vi "ControllerUI_New - 副本.vi"() -> ()   [LabVIEW 2026]
uses:
  <vilib>/Utility/error.llb/Trim Whitespace One-Sided.vi
panel:
  in  "Tab Control":T1(tab)
  out "background 2":picture
  in  "5-Day Rainstorm-to-Flood":bool
  out "script Status":string
  in  "voltage 1":dbl
  in  "DESD4 SOC":dbl(slide) step=1.0 scale=0.0..100.0 scale format="%#.6g"
  in  "DESD3 SOC":dbl(slide) step=1.0 scale=0.0..100.0 scale format="%#.6g"
  in  "DESD2 SOC":dbl(slide) step=1.0 scale=0.0..100.0 scale format="%#.6g"
  in  "wind speed":dbl(knob) caption="Wind Speed (m/s)" min=0.0 max=30.0 step=0.5 scale=0.0..255.0
  in  "stop":bool
  in  "Send UDP Command":bool caption="IO Building Send"
  out "Device Badge":string
  out "Selected Summary":string
  out "Device Description":string
  out "Device Name":string
  in  "DESD1 SOC":dbl(slide) step=1.0 scale=0.0..100.0 scale format="%#.6g"
  in  "BTN_DESD_4":bool
  in  "BTN_PV_1":bool
  in  "BTN_DESD_2":bool
  in  "BTN_Gen_1":bool
  in  "BTN_DESD_1":bool
  in  "BTN_Gen_2":bool
  in  "BTN_DESD_3":bool
  in  "BTN_PV_2":bool
  in  "BTN_Load_2":bool
  in  "BTN_Load_4":bool
  in  "BTN_Grid_1":bool
  in  "BTN_Load_3":bool
  in  "BTN_Wind_Turbine":bool
  out "background":picture
  in  "IO 1":bool
  in  "IO 2":bool
  in  "IO 3":bool
  in  "IO 4":bool
  in  "IO 6":bool
  in  "IO 7":bool
  in  "IO 8":bool
  in  "IO 5":bool
  in  "IO 9":bool
  in  "IO 10":bool
  in  "IO 11":bool
  in  "IO 12":bool
  in  "IO 13":bool
  in  "IO 14":bool
  in  "IO 15":bool
  in  "IO 16":bool
  in  "voltage 2":dbl
  in  "voltage 3":dbl
  in  "voltage 4":dbl
  # "LabVIEW-Based Physical Sandbox Intelligent Control System"
  # "LabVIEW-Based Physical Sandbox Intelligent Control System"
  # "Node Information"
  # "Control Panel"
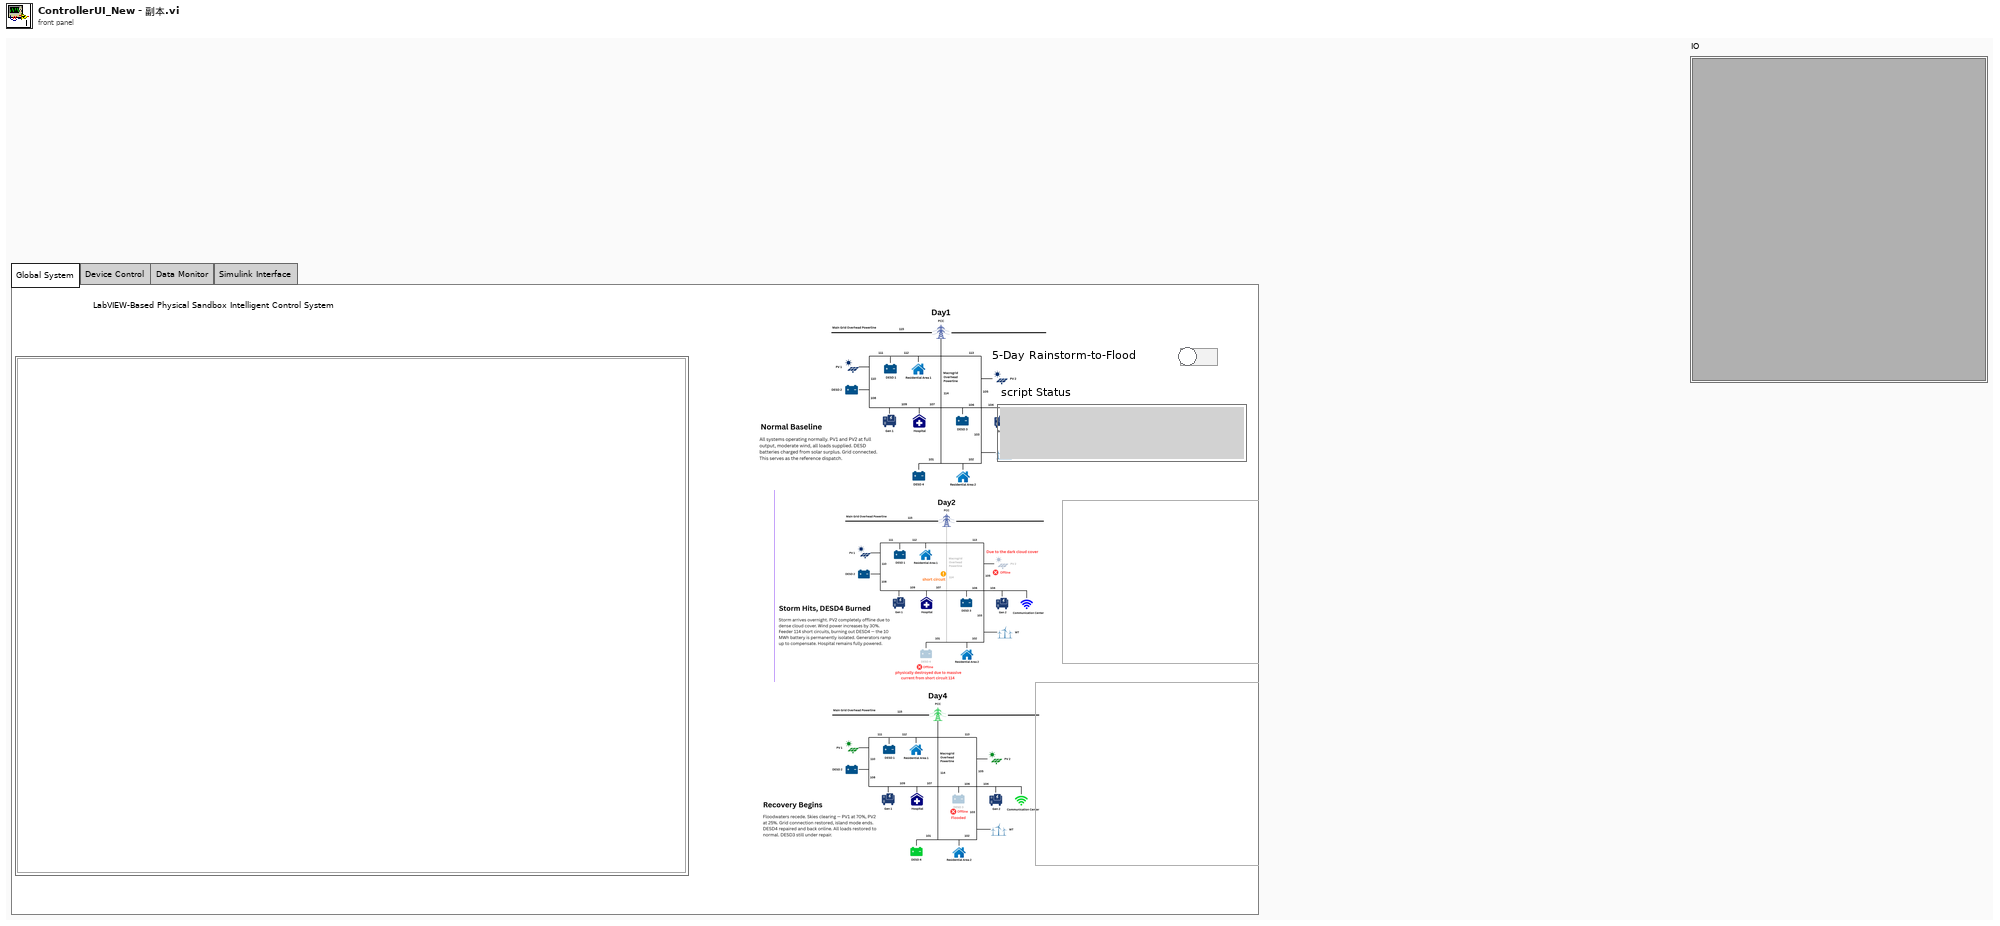
[diagram p1: front panel]
types:
  T1 = enum32{"Global System", "Device Control", "Data Monitor", "Simulink Interface"}
  T2 = typedef "imagedata.ctl" = cluster{"image type":i32, "image depth":i32, "image":u8[], "mask":u8[], "colors":u32[], "Rectangle":cluster{"left":i16, "top":i16, "right":i16, "bottom":i16}}
  T3 = cluster{string, "wind speed":dbl, i32, i32, i32, i32}
  T4 = cluster{string, " DESD4 SOC":dbl, dbl, dbl, i32, i32}
  T5 = cluster{string, " DESD3 SOC":dbl, dbl, dbl, i32, i32}
  T6 = cluster{string, " DESD2 SOC":dbl, dbl, dbl, i32, i32}
  T7 = cluster{string, " DESD1 SOC":dbl, dbl, dbl, i32, i32}
  T8 = cluster{string, " DESD4 SOC":dbl, dbl, dbl, i32, i32}[]
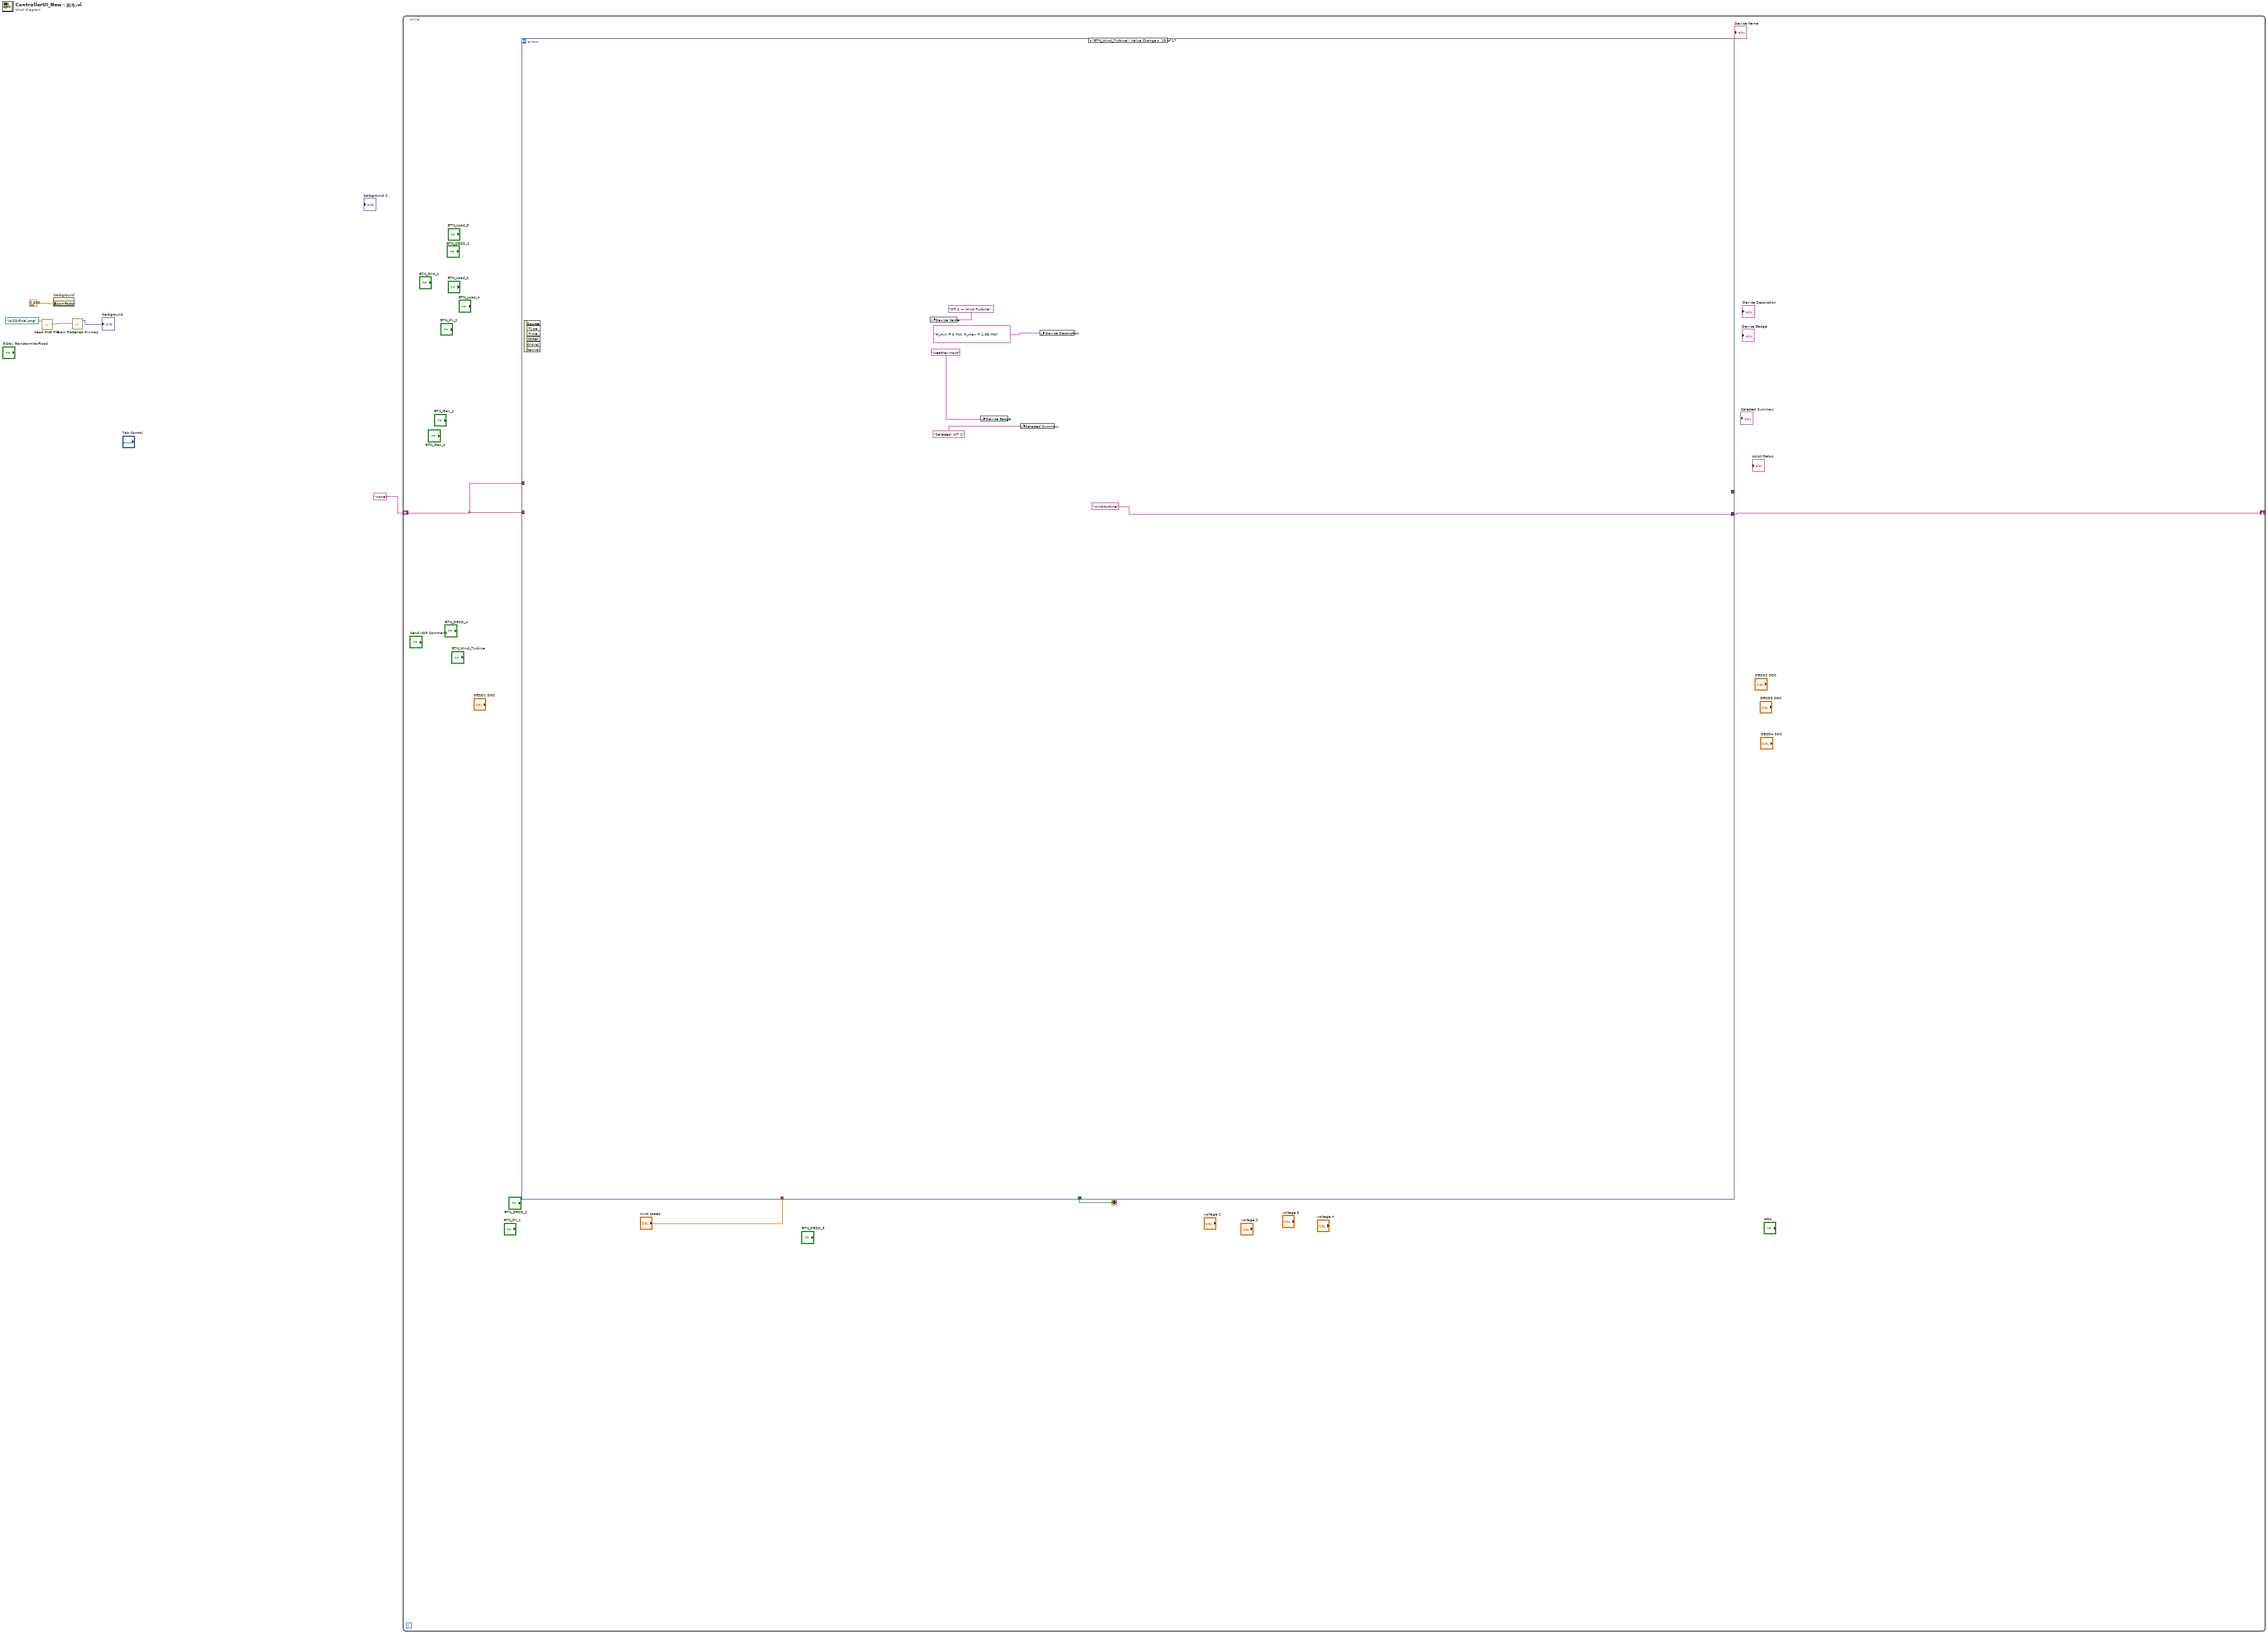
[diagram p0: block diagram]
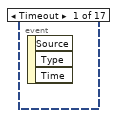
[diagram p2: hidden frame]
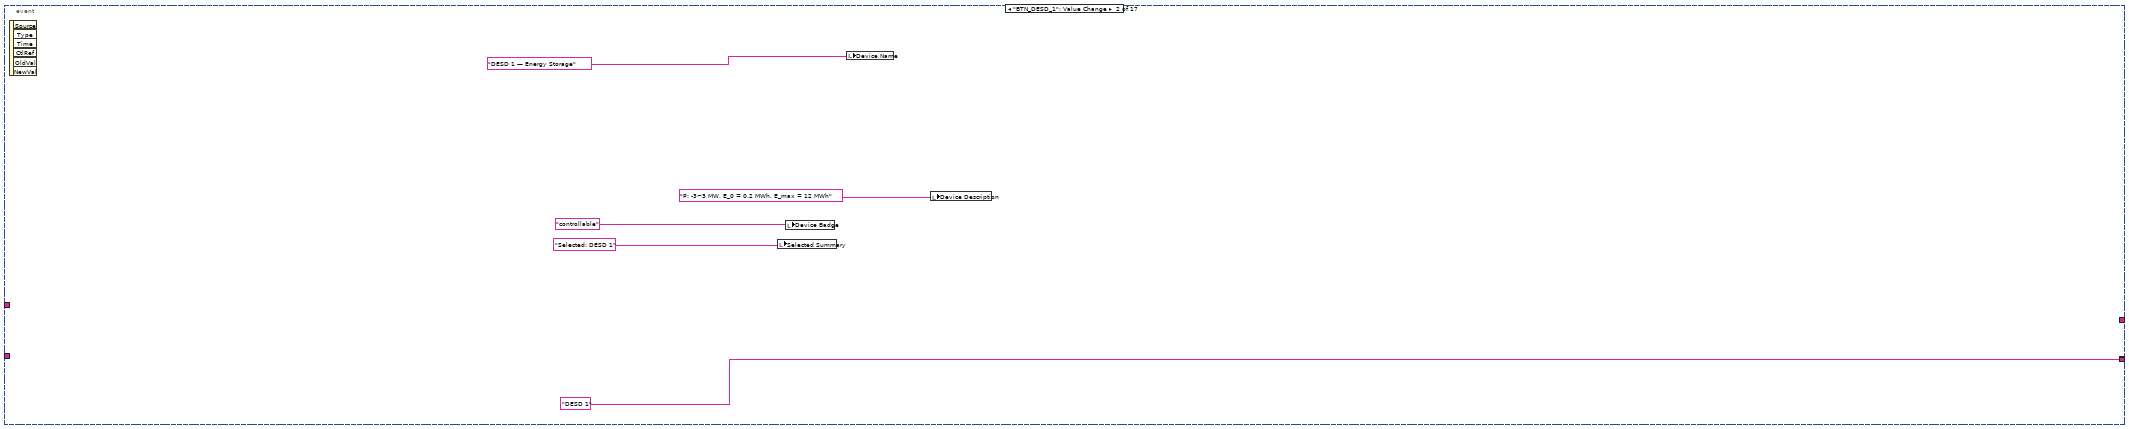
[diagram p3: hidden frame]
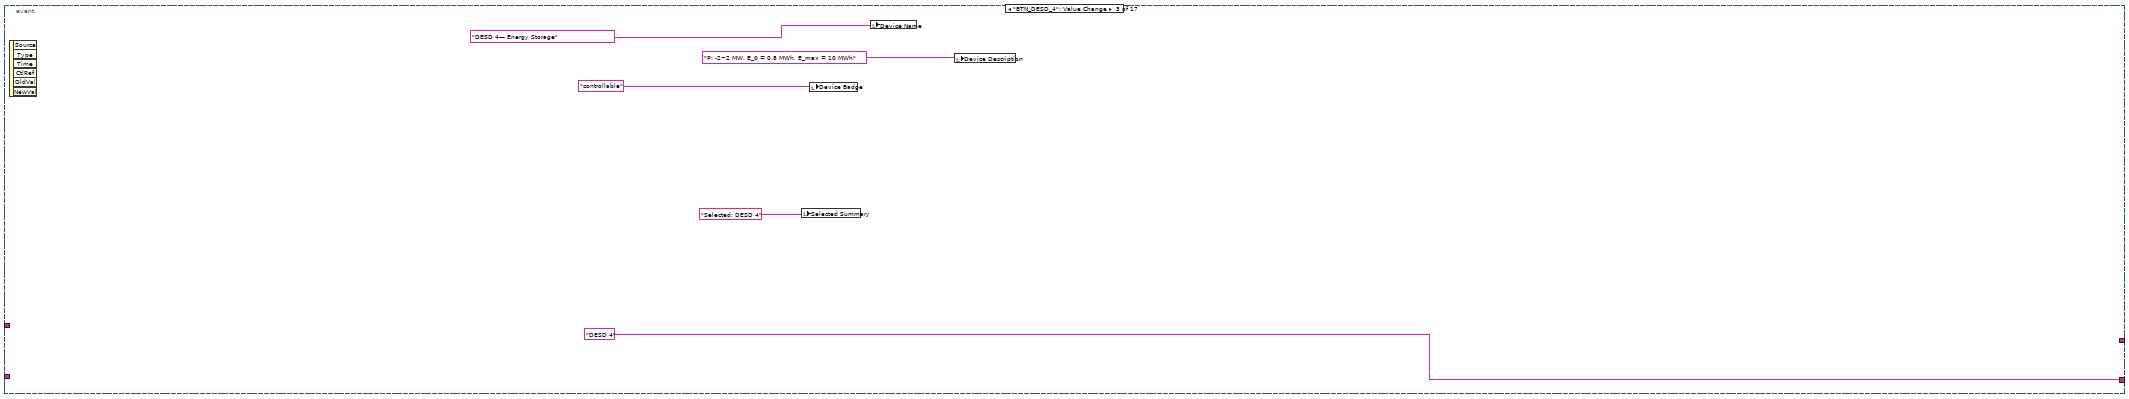
[diagram p4: hidden frame]
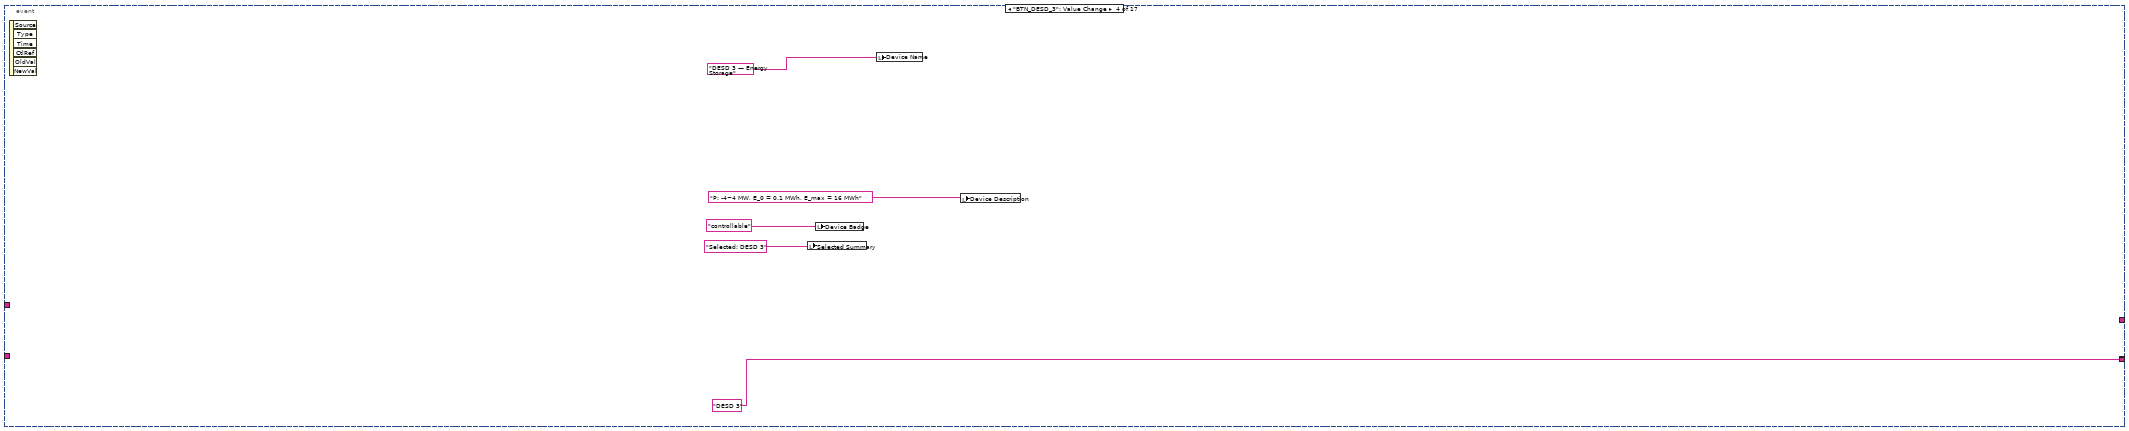
[diagram p5: hidden frame]
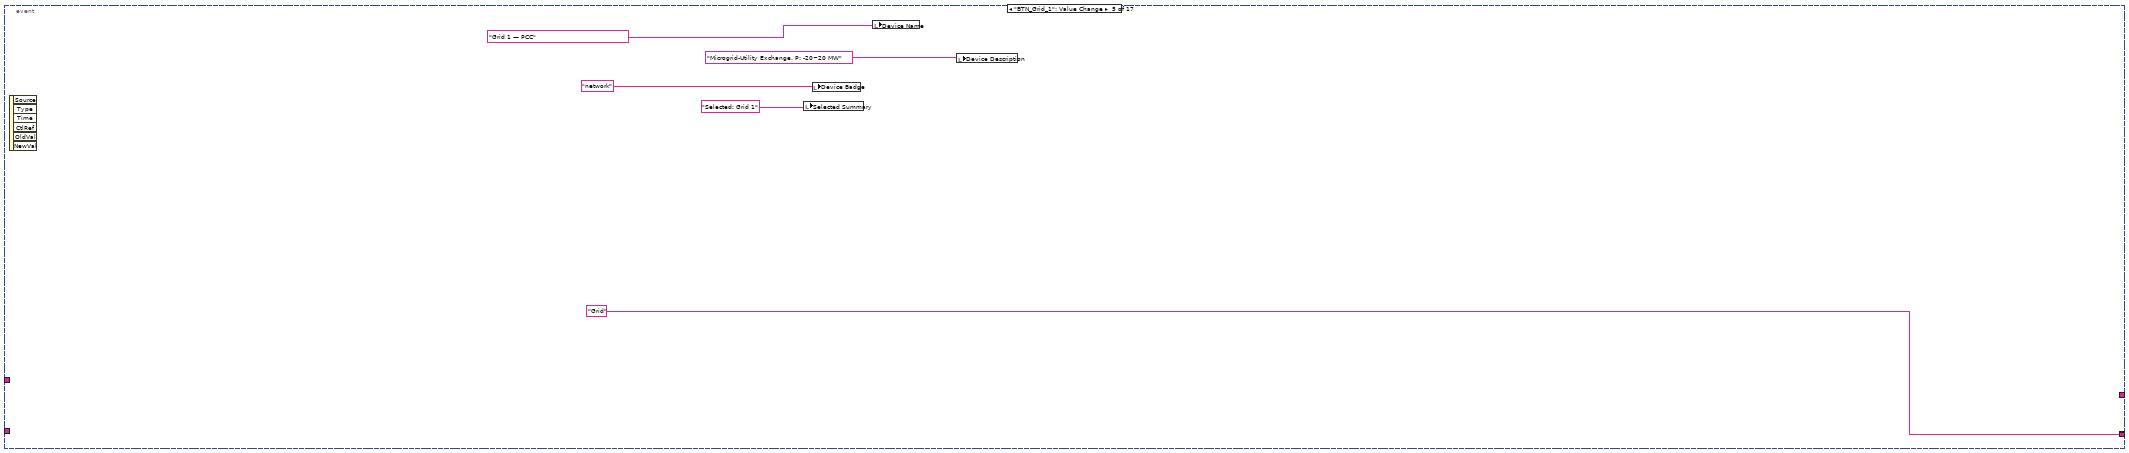
[diagram p6: hidden frame]
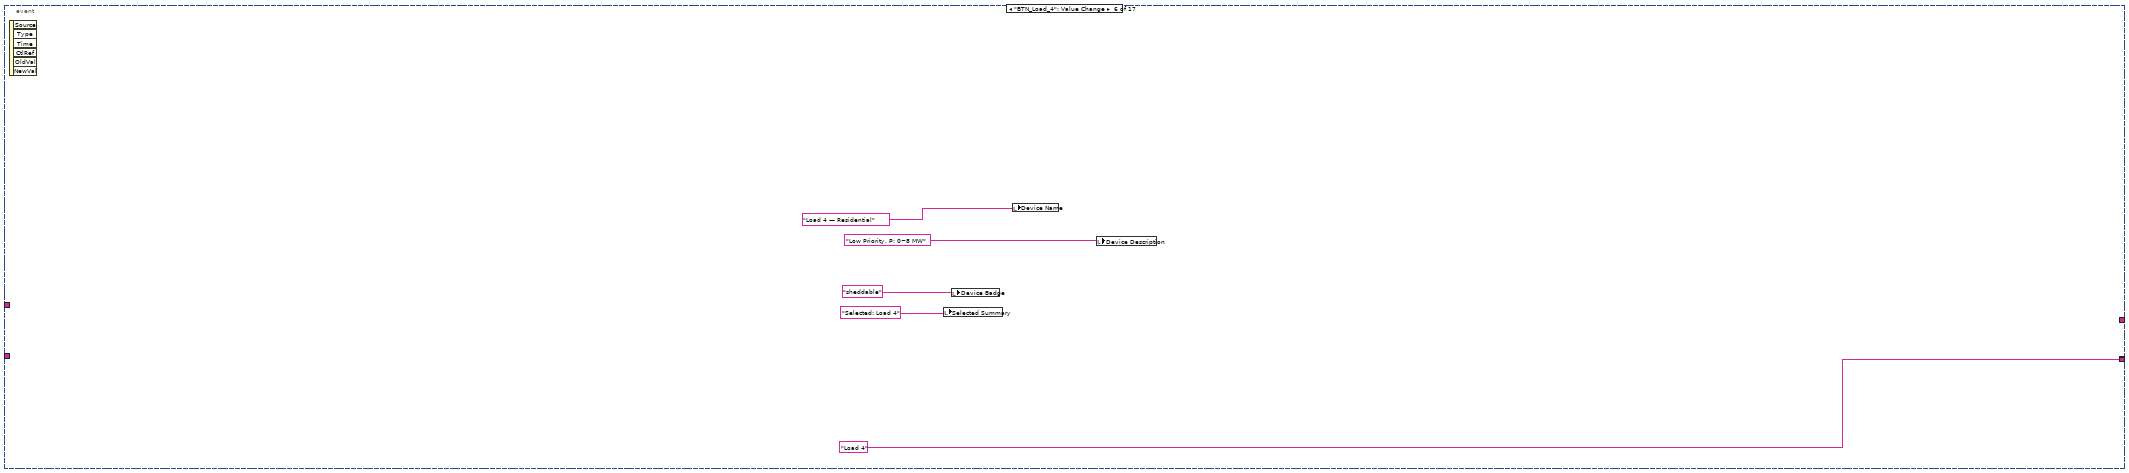
[diagram p7: hidden frame]
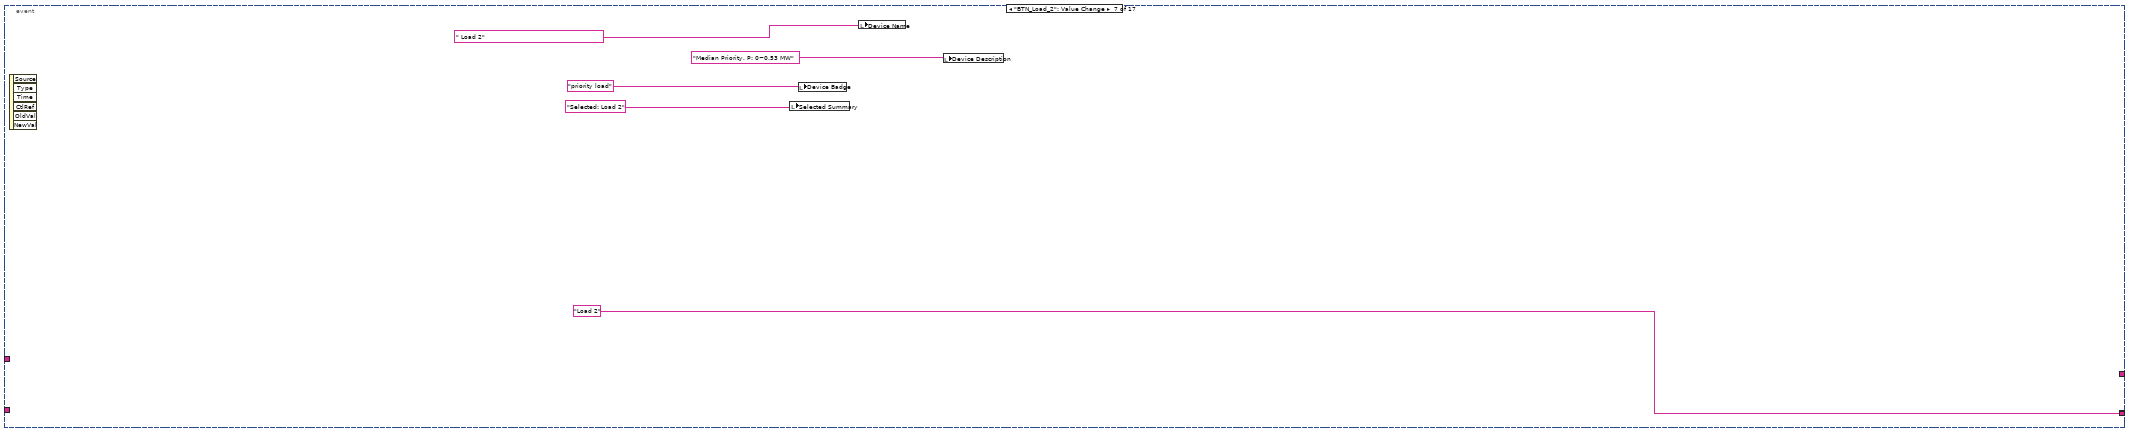
[diagram p8: hidden frame]
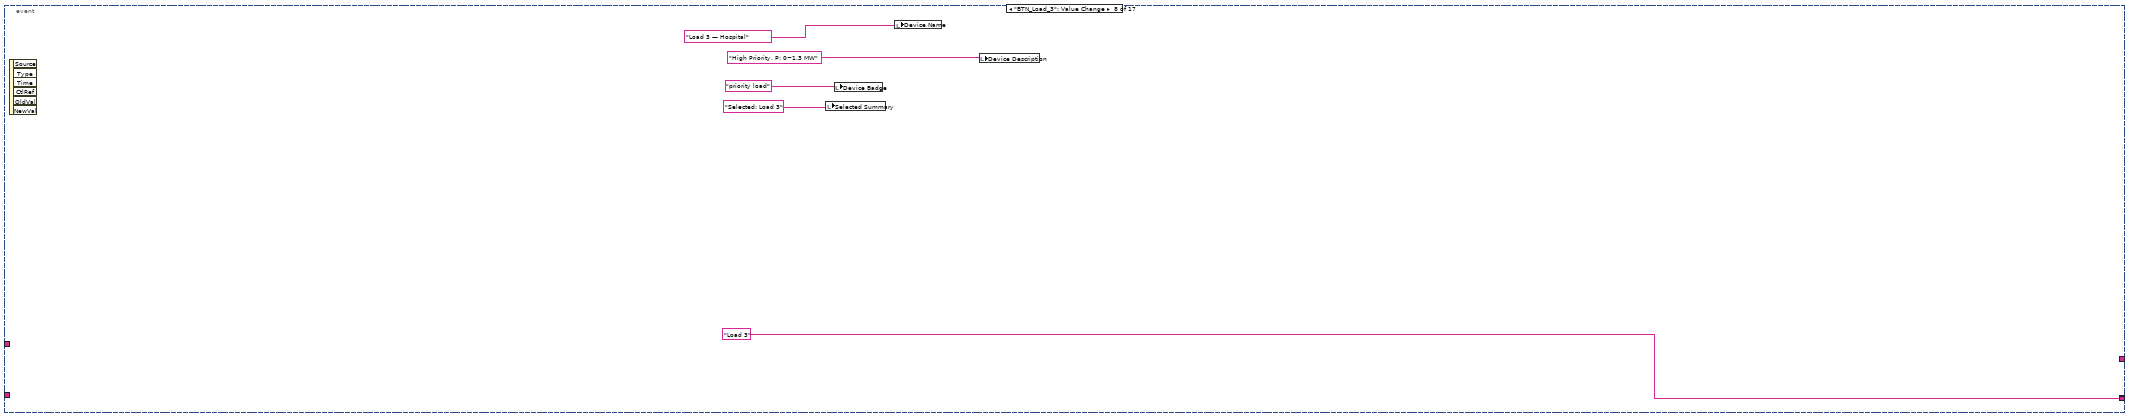
[diagram p9: hidden frame]
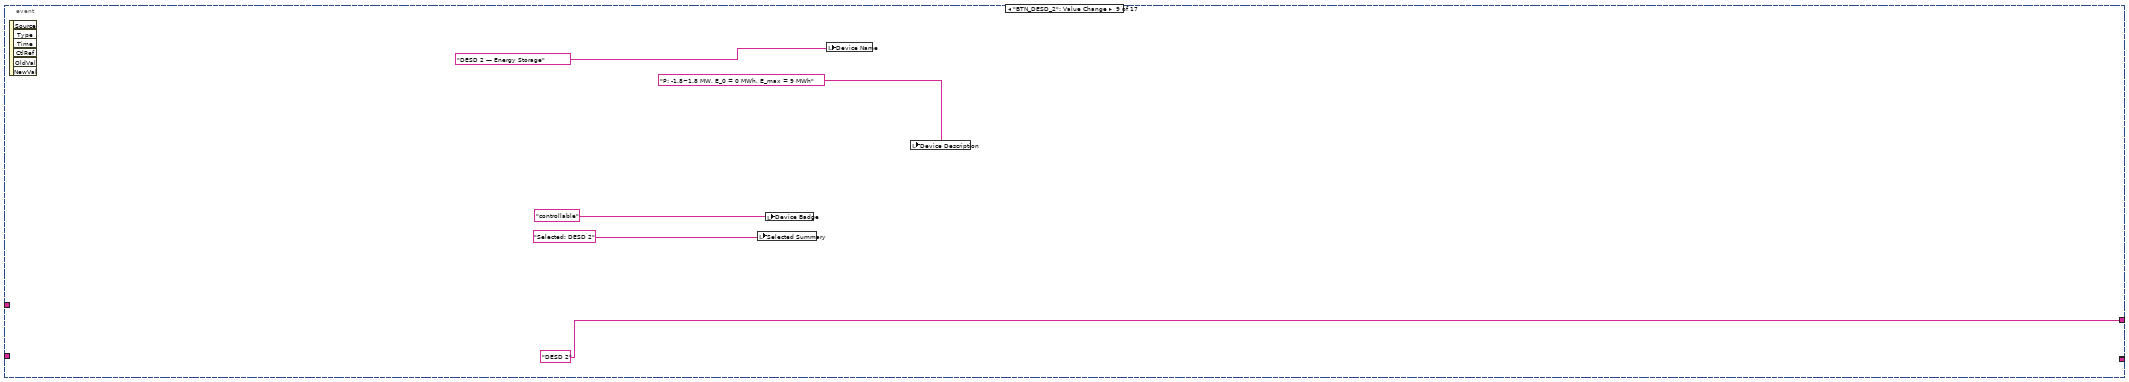
[diagram p10: hidden frame]
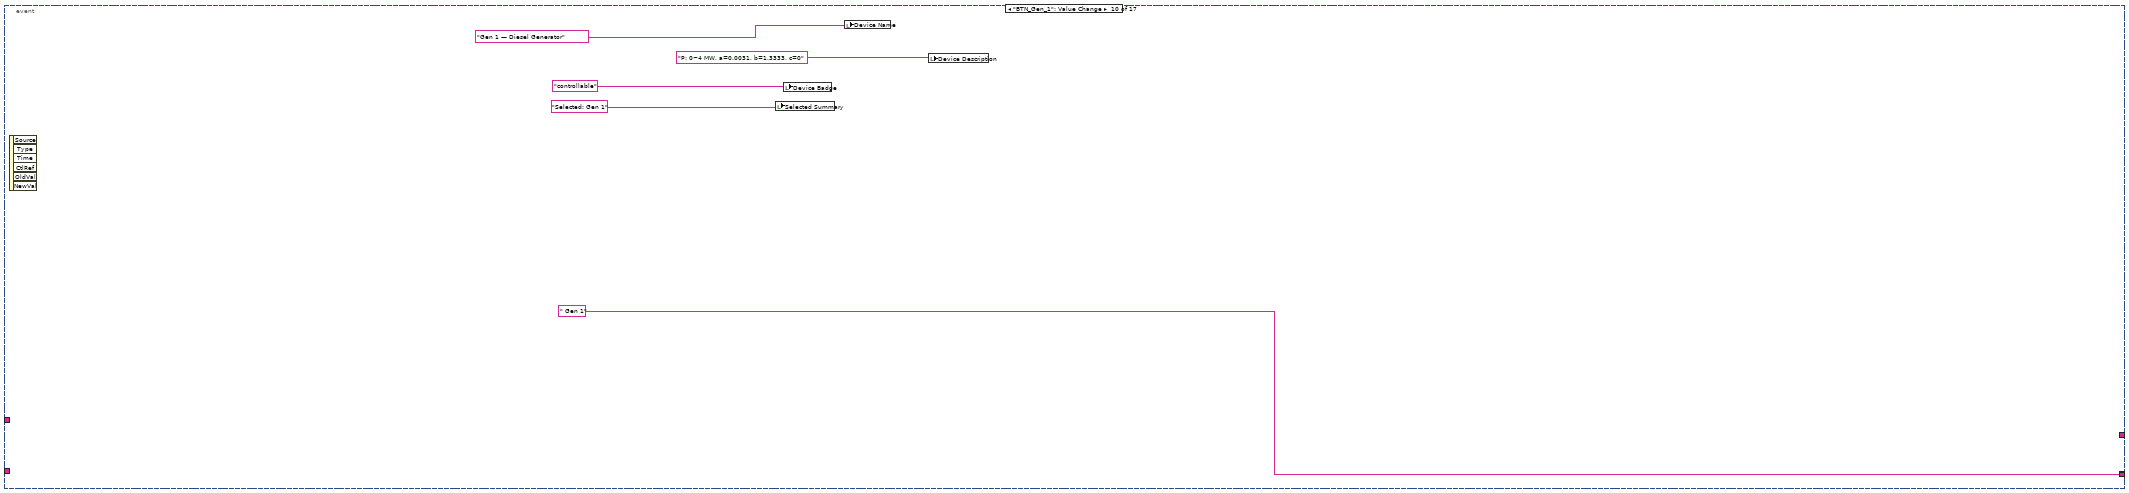
[diagram p11: hidden frame]
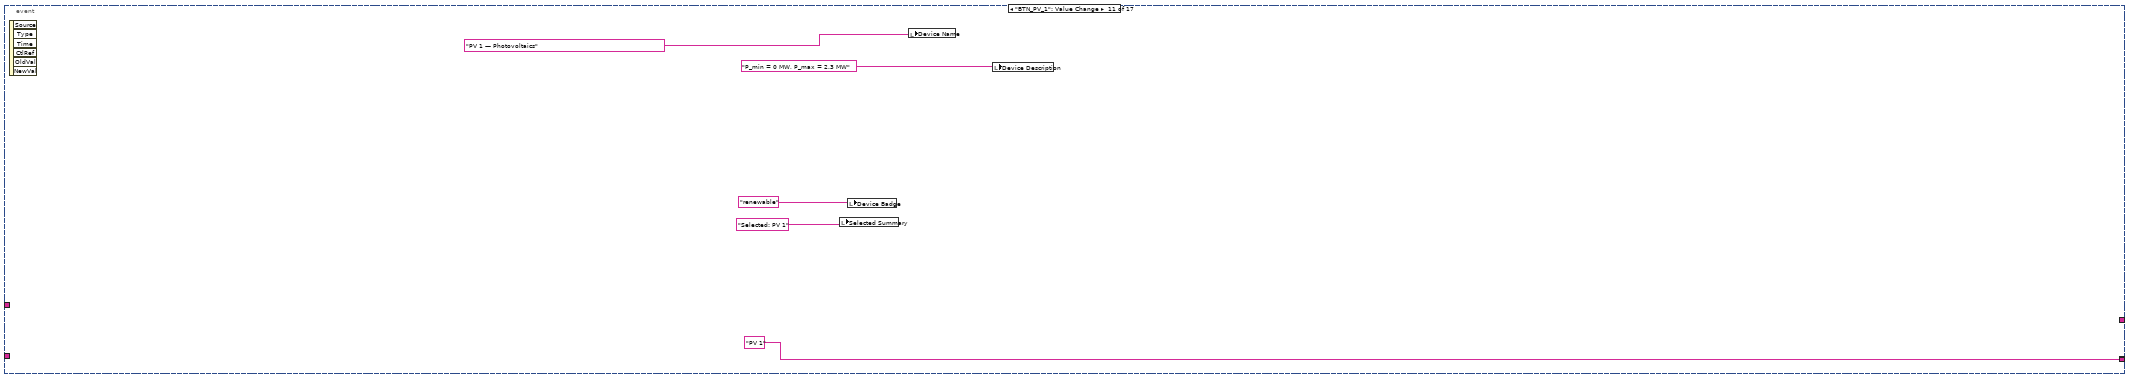
[diagram p12: hidden frame]
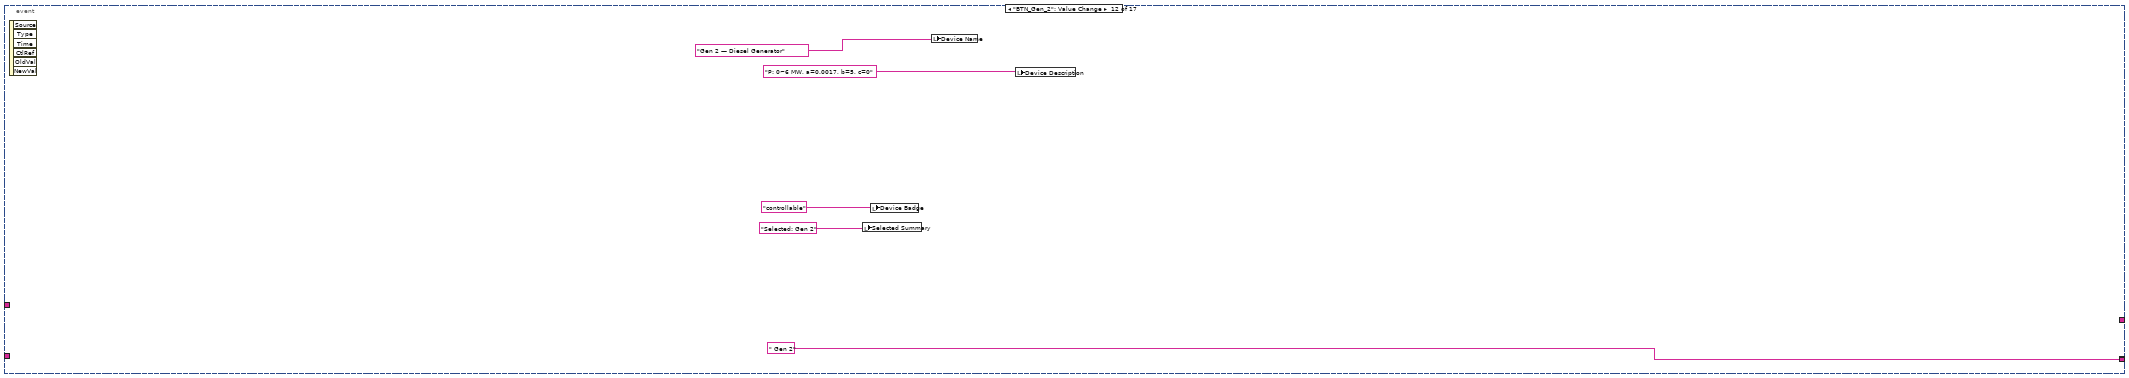
[diagram p13: hidden frame]
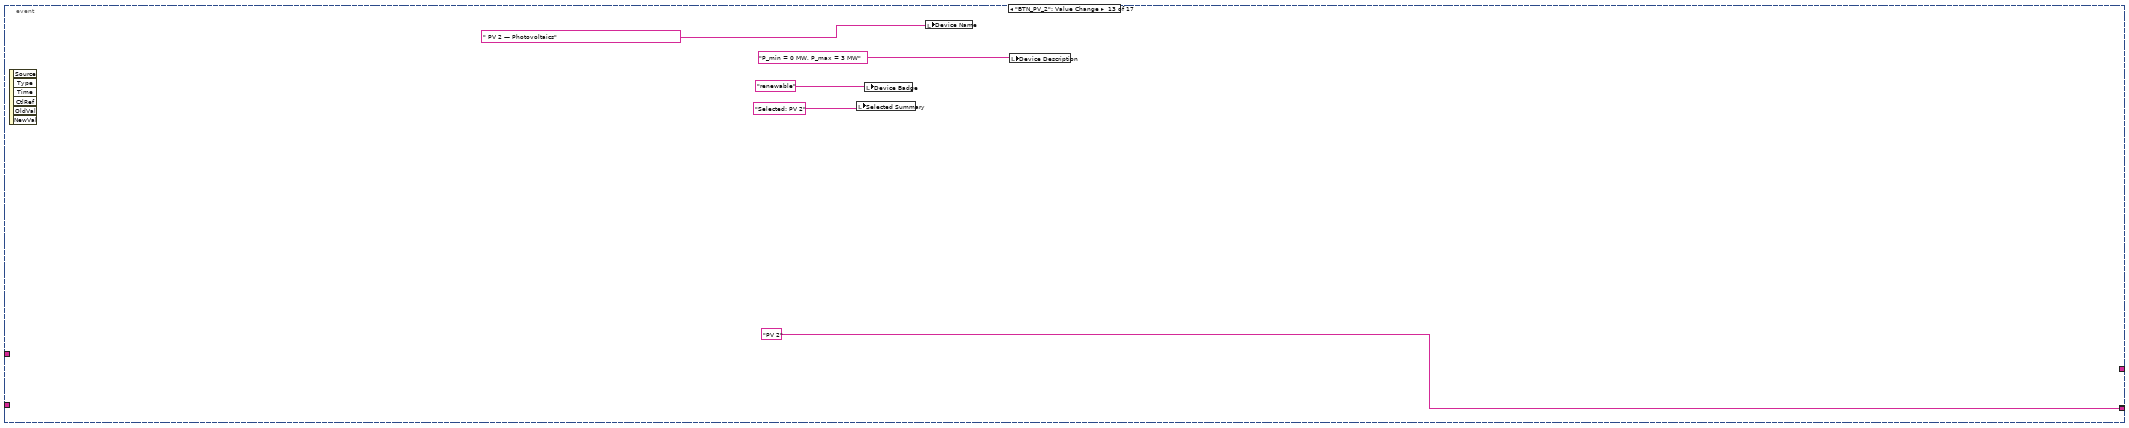
[diagram p14: hidden frame]
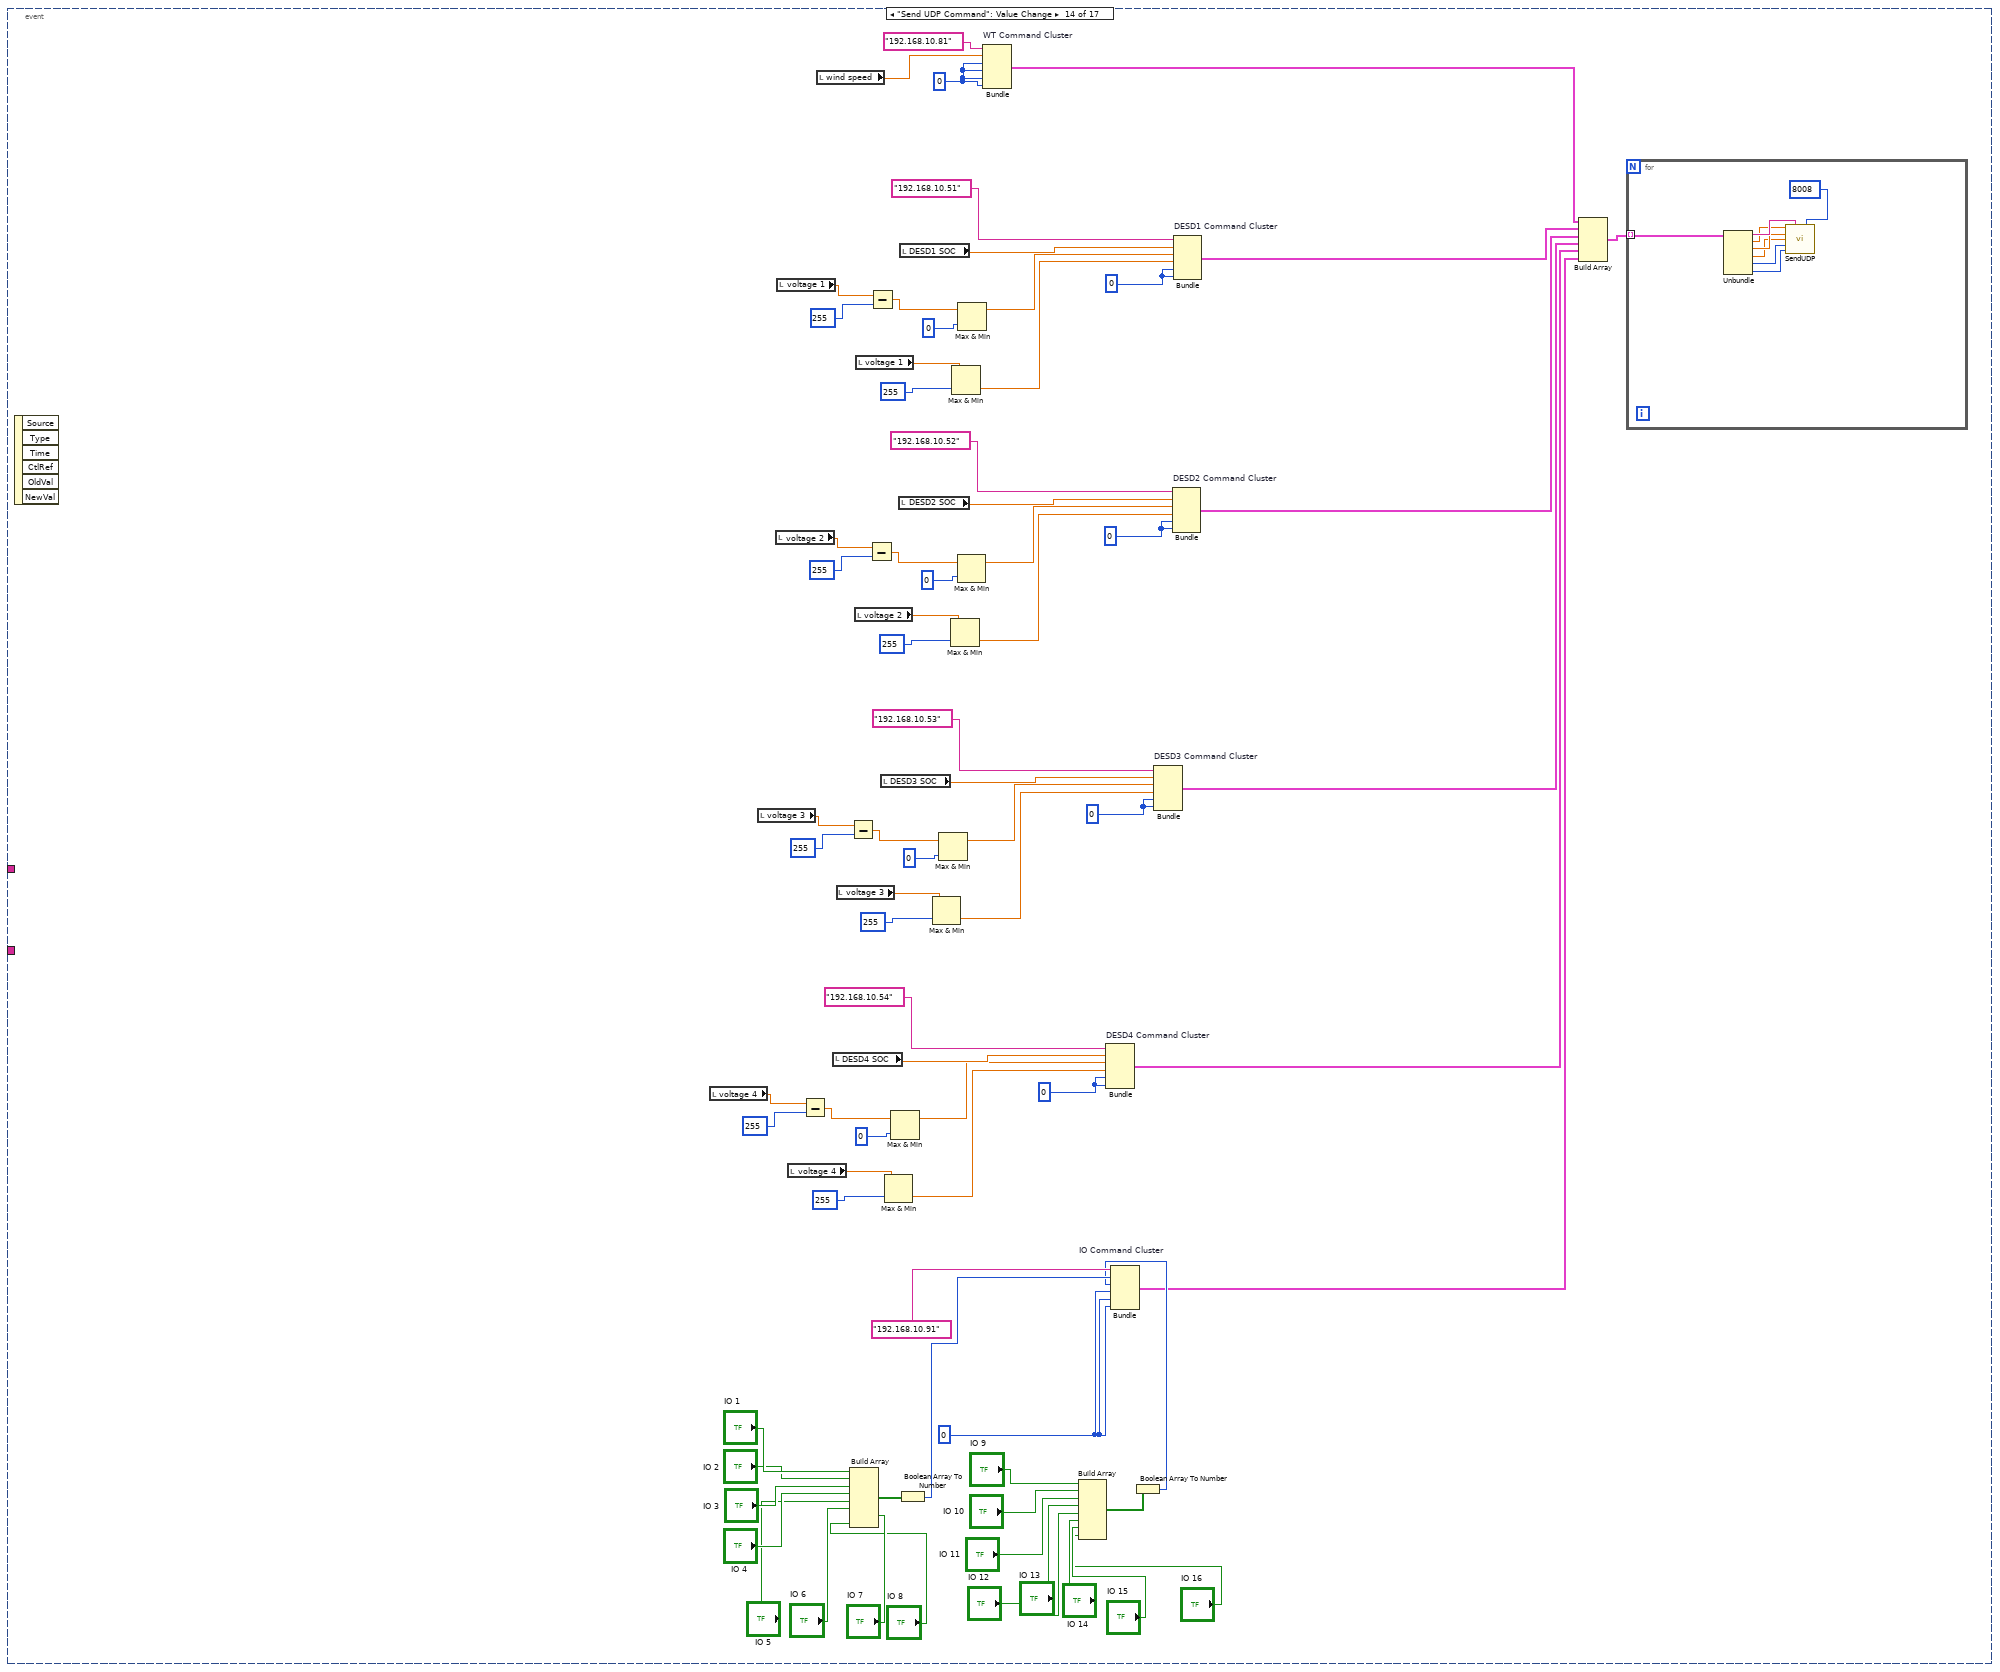
[diagram p15: hidden frame]
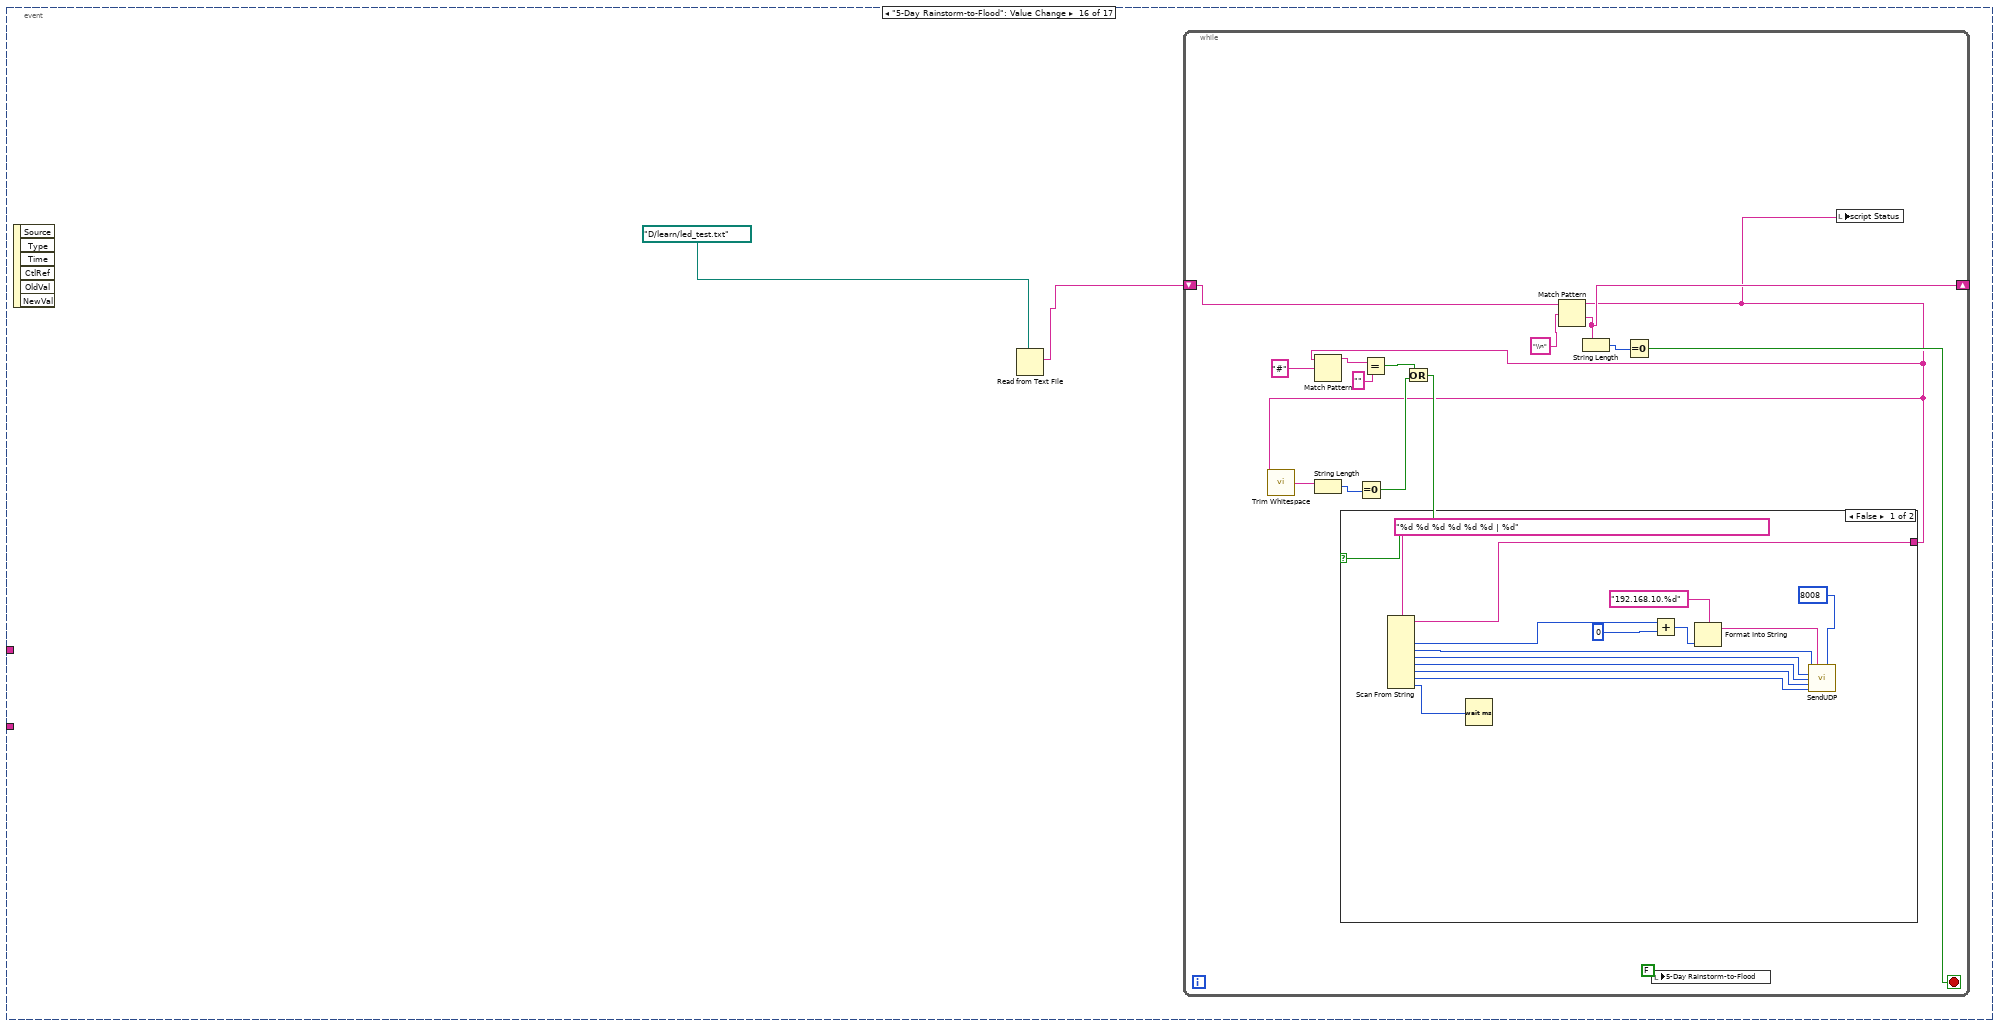
[diagram p16: hidden frame]
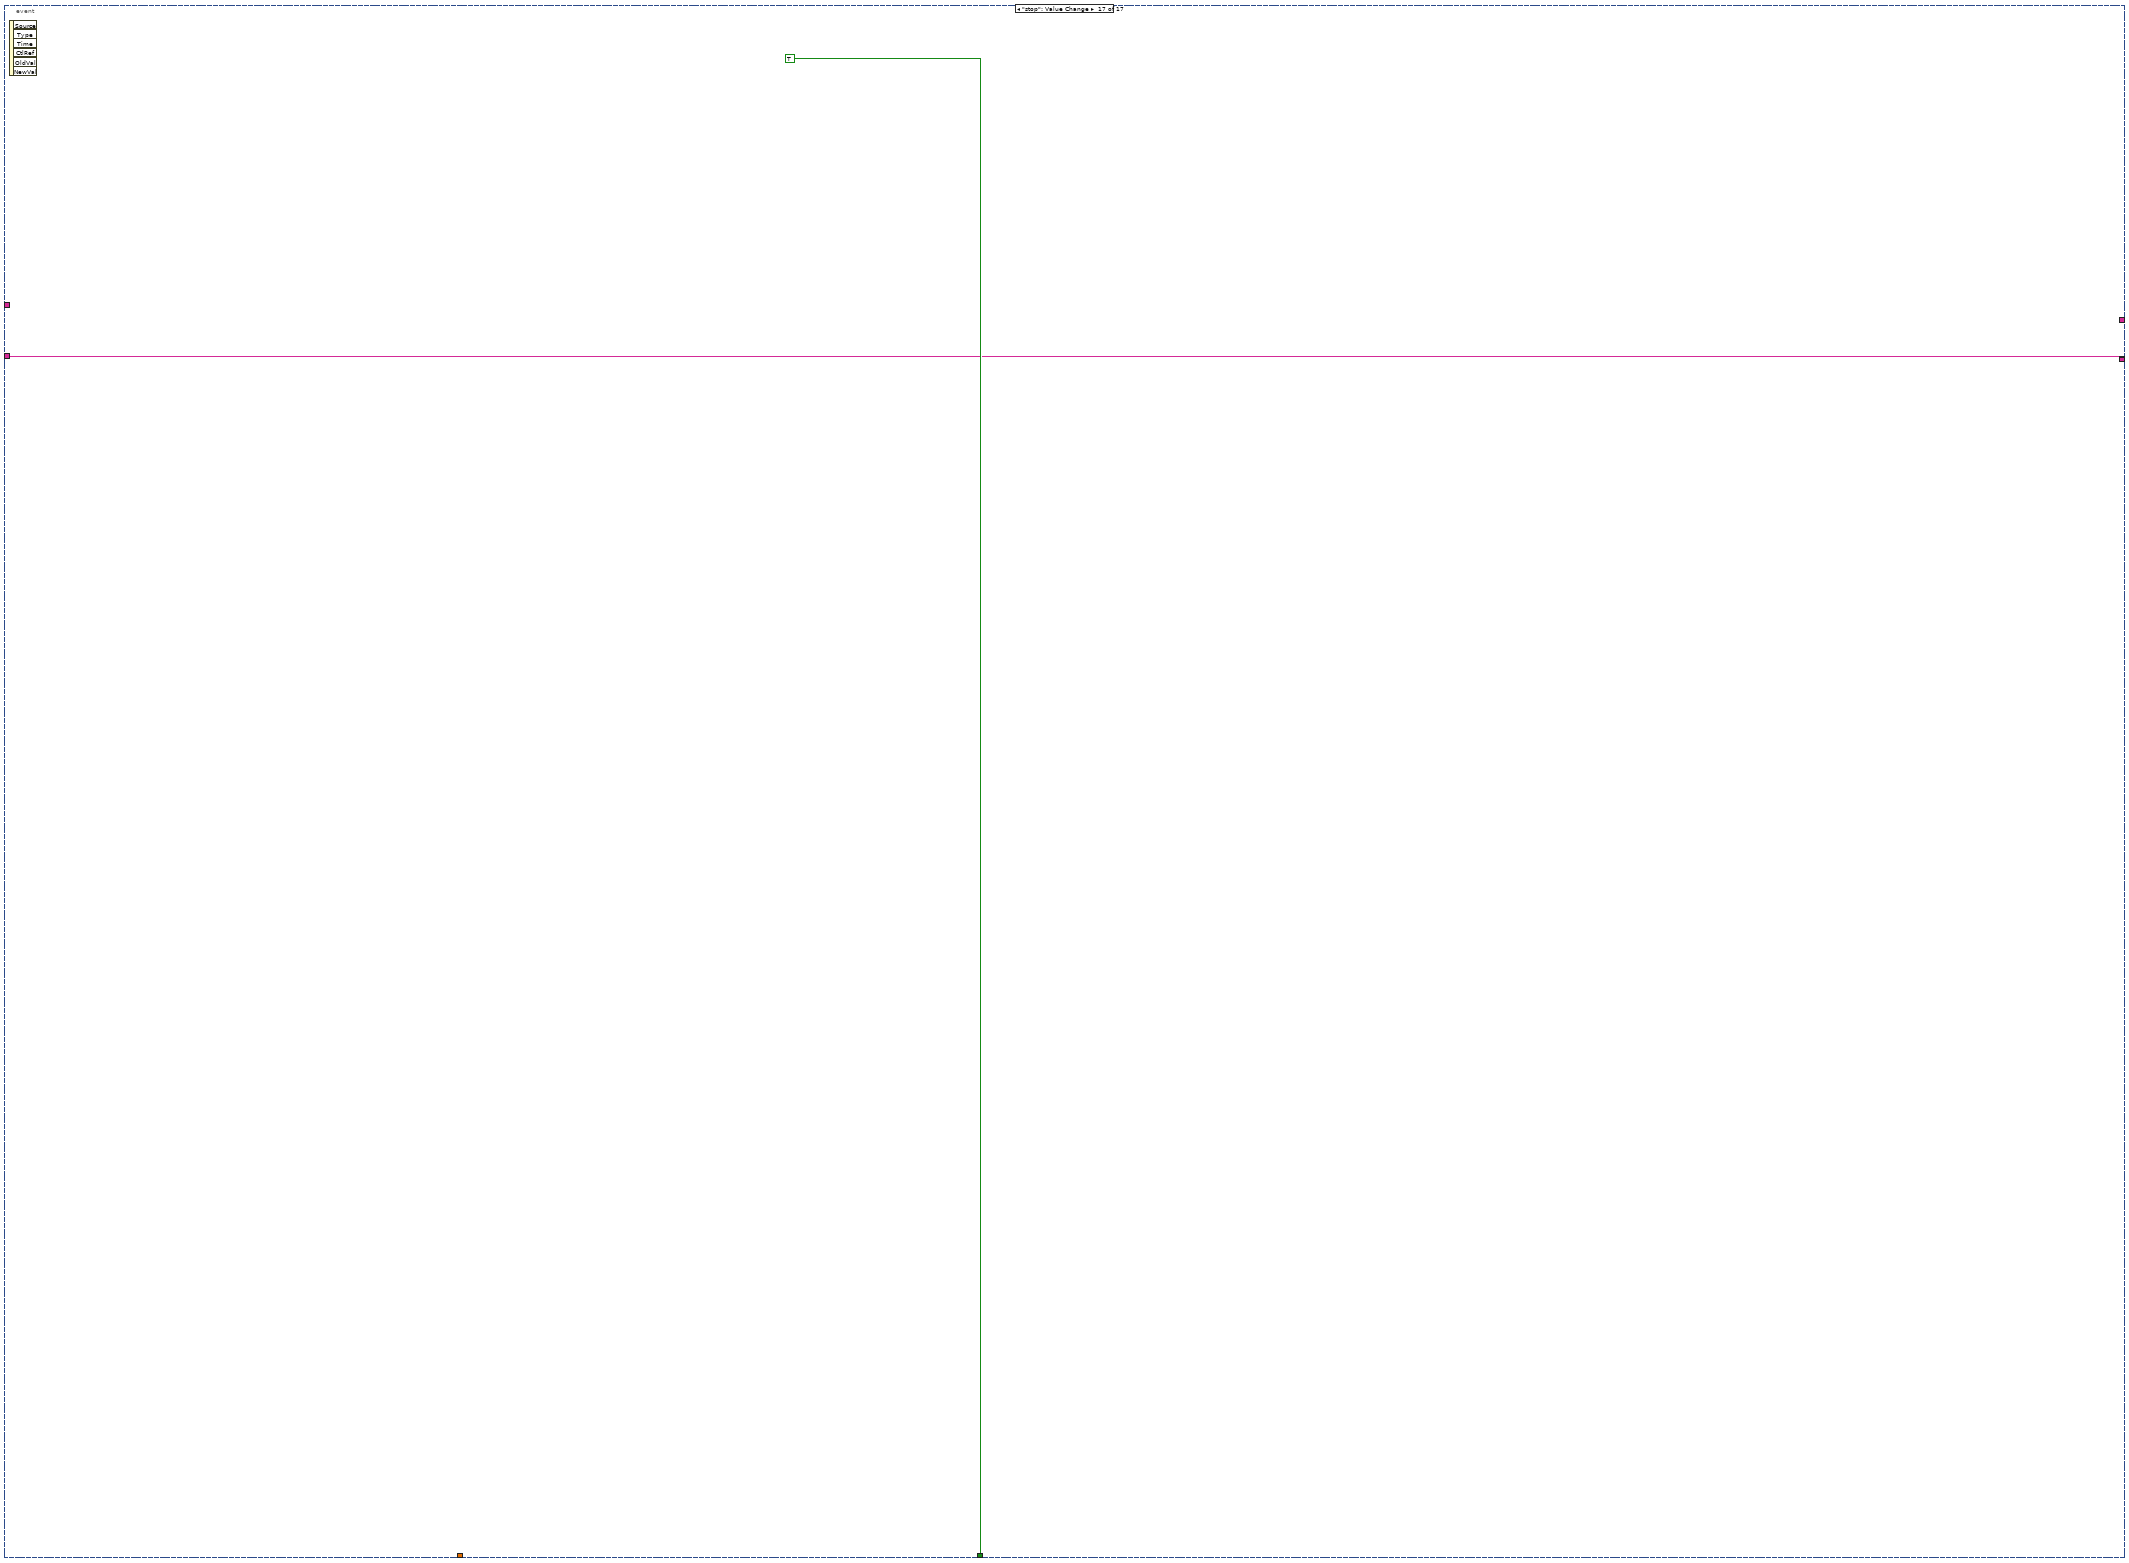
[diagram p18: hidden frame]
diagram:
  n1 = call <vilib>:"Read PNG File.vi"("path to PNG file"=path "ip-2D-final.png") -> ("image data"=w5:T2)  [unwired: 8 in, 2 out]
  n2 = property on="background" class="Pict"("ZoomFactor"=sgl 0.6 ("Zoom Factor")) -> ()  [unwired: 2 in, 2 out]
  n3 = call <vilib>:"Draw Flattened Pixmap.vi"("image data"=w5) -> ("new picture"=→"background":picture)  [unwired: 8 in]
  n4 = while {
    shift-right: [w7] -> _
    shift-left: "none" -> [w6]
    stop <- w9 stop-if-true
    n5 = event shown="[14] \"BTN_Wind_Turbine\": Value Change" {
      selector: _ -> [_ _ _ _ _ _ _ _ _ _ _ _ _ _ _ _ _]
      dyn-events: _ -> [_ _ _ _ _ _ _ _ _ _ _ _ _ _ _ _ _]
      timeout: _ -> [_ _ _ _ _ _ _ _ _ _ _ _ _ _ _ _ _]
      tunnel: [_ _ _ _ _ _ _ _ _ _ _ _ _ _ _ _ TRUE] -> w9
      tunnel: [_ _ _ _ _ _ _ _ "DESD 2" _ _ _ _ _ _ _ _] -> _
      tunnel: "wind speed" -> [_ _ _ _ _ _ _ _ _ _ _ _ _ _ _ _ _]
      tunnel: [_ "DESD 1" "DESD 4" "DESD 3" "Grid" "Load 4" "Load 2" "Load 3" _ " Gen 1" "PV 1" " Gen 2" _ _ "wind-turbine" _ w190] -> w7
      tunnel: w6 -> [_ _ _ _ _ _ _ _ _ _ _ _ _ _ _ _ _]
      tunnel: w6 -> [_ _ _ _ _ _ _ _ _ _ _ _ _ _ _ _ w190]
      tunnel: [_ _ _ _ _ _ _ _ _ _ _ _ "PV 2" _ _ _ _] -> _
      event Timeout {
        n6 = event-data() -> ()  [unwired: 1 in, 3 out]
      }
      event "BTN_DESD_1": Value Change {
        n7 = event-data() -> ()  [unwired: 1 in, 6 out]
        n8 = local write "Selected Summary"("Selected: DESD 1") -> ()
        n9 = local write "Device Badge"("controllable") -> ()
        n10 = local write "Device Name"("DESD 1 — Energy Storage") -> ()
        n11 = local write "Device Description"("P: -3~3 MW, E_0 = 0.2 MWh, E_max = 12 MWh") -> ()
      }
      event "BTN_DESD_4": Value Change {
        n12 = event-data() -> ()  [unwired: 1 in, 6 out]
        n13 = local write "Selected Summary"("Selected: DESD 4") -> ()
        n14 = local write "Device Badge"("controllable") -> ()
        n15 = local write "Device Name"("DESD 4— Energy Storage") -> ()
        n16 = local write "Device Description"("P: -2~2 MW, E_0 = 0.8 MWh, E_max = 10 MWh") -> ()
      }
      event "BTN_DESD_3": Value Change {
        n17 = event-data() -> ()  [unwired: 1 in, 6 out]
        n18 = local write "Selected Summary"("Selected: DESD 3") -> ()
        n19 = local write "Device Badge"("controllable") -> ()
        n20 = local write "Device Name"("DESD 3 — Energy Storage") -> ()
        n21 = local write "Device Description"("P: -4~4 MW, E_0 = 0.1 MWh, E_max = 16 MWh") -> ()
      }
      event "BTN_Grid_1": Value Change {
        n22 = event-data() -> ()  [unwired: 1 in, 6 out]
        n23 = local write "Selected Summary"("Selected: Grid 1") -> ()
        n24 = local write "Device Badge"("network") -> ()
        n25 = local write "Device Name"("Grid 1 — PCC") -> ()
        n26 = local write "Device Description"("Microgrid-Utility Exchange. P: -20~20 MW") -> ()
      }
      event "BTN_Load_4": Value Change {
        n27 = event-data() -> ()  [unwired: 1 in, 6 out]
        n28 = local write "Selected Summary"("Selected: Load 4") -> ()
        n29 = local write "Device Badge"("sheddable") -> ()
        n30 = local write "Device Name"("Load 4 — Residential") -> ()
        n31 = local write "Device Description"("Low Priority. P: 0~8 MW") -> ()
      }
      event "BTN_Load_2": Value Change {
        n32 = event-data() -> ()  [unwired: 1 in, 6 out]
        n33 = local write "Selected Summary"("Selected: Load 2") -> ()
        n34 = local write "Device Badge"("priority load") -> ()
        n35 = local write "Device Name"(" Load 2") -> ()
        n36 = local write "Device Description"("Median Priority. P: 0~0.53 MW") -> ()
      }
      event "BTN_Load_3": Value Change {
        n37 = event-data() -> ()  [unwired: 1 in, 6 out]
        n38 = local write "Selected Summary"("Selected: Load 3") -> ()
        n39 = local write "Device Badge"("priority load") -> ()
        n40 = local write "Device Name"("Load 3 — Hospital") -> ()
        n41 = local write "Device Description"("High Priority. P: 0~1.3 MW") -> ()
      }
      event "BTN_DESD_2": Value Change {
        n42 = event-data() -> ()  [unwired: 1 in, 6 out]
        n43 = local write "Selected Summary"("Selected: DESD 2") -> ()
        n44 = local write "Device Badge"("controllable") -> ()
        n45 = local write "Device Name"("DESD 2 — Energy Storage") -> ()
        n46 = local write "Device Description"("P: -1.8~1.8 MW, E_0 = 0 MWh, E_max = 9 MWh") -> ()
      }
      event "BTN_Gen_1": Value Change {
        n47 = event-data() -> ()  [unwired: 1 in, 6 out]
        n48 = local write "Selected Summary"("Selected: Gen 1") -> ()
        n49 = local write "Device Badge"("controllable") -> ()
        n50 = local write "Device Name"("Gen 1 — Diesel Generator") -> ()
        n51 = local write "Device Description"("P: 0~4 MW, a=0.0031, b=1.3333, c=0") -> ()
      }
      event "BTN_PV_1": Value Change {
        n52 = event-data() -> ()  [unwired: 1 in, 6 out]
        n53 = local write "Selected Summary"("Selected: PV 1") -> ()
        n54 = local write "Device Badge"("renewable") -> ()
        n55 = local write "Device Name"("PV 1 — Photovoltaics") -> ()
        n56 = local write "Device Description"("P_min = 0 MW, P_max = 2.3 MW") -> ()
      }
      event "BTN_Gen_2": Value Change {
        n57 = event-data() -> ()  [unwired: 1 in, 6 out]
        n58 = local write "Selected Summary"("Selected: Gen 2") -> ()
        n59 = local write "Device Badge"("controllable") -> ()
        n60 = local write "Device Name"("Gen 2 — Diesel Generator") -> ()
        n61 = local write "Device Description"("P: 0~6 MW, a=0.0017, b=5, c=0") -> ()
      }
      event "BTN_PV_2": Value Change {
        n62 = event-data() -> ()  [unwired: 1 in, 6 out]
        n63 = local write "Selected Summary"("Selected: PV 2") -> ()
        n64 = local write "Device Badge"("renewable") -> ()
        n65 = local write "Device Name"(" PV 2 — Photovoltaics") -> ()
        n66 = local write "Device Description"("P_min = 0 MW, P_max = 3 MW") -> ()
      }
      event "Send UDP Command": Value Change {
        w81 = 0
        w92 = 0
        w103 = 0
        w114 = 0
        w126 = 0
        w77 = 0
        n67 = event-data() -> ()  [unwired: 1 in, 6 out]
        n68 = local read "voltage 4"() -> (w88:dbl)
        n69 = local read "voltage 3"() -> (w99:dbl)
        n70 = local read "voltage 2"() -> (w110:dbl)
        n71 = local read "voltage 1"() -> (w121:dbl)
        n72 = local read "voltage 4"() -> (w91:dbl)
        n73 = Subtract(x=w88, y=255) -> (x-y=w86:dbl)
        n74 = local read "wind speed"() -> (w125:dbl)
        n75 = local read "DESD4 SOC"() -> (w84:dbl)
        n76 = local read "voltage 3"() -> (w102:dbl)
        n77 = Subtract(x=w99, y=255) -> (x-y=w97:dbl)
        n78 = Build Array("IO 1", "IO 2", "IO 3", "IO 4", "IO 5", "IO 6", "IO 7", "IO 8") -> (w129:bool[])
        n79 = local read "voltage 2"() -> (w113:dbl)
        n80 = local read "voltage 1"() -> (w124:dbl)
        n81 = Subtract(x=w110, y=255) -> (x-y=w108:dbl)
        n82 = Subtract(x=w121, y=255) -> (x-y=w119:dbl)
        n83 = local read "DESD3 SOC"() -> (w95:dbl)
        n84 = Max & Min(x=w91, y=255) -> (min(x,y)=w82:dbl)  [unwired: 1 out]
        n85 = Max & Min(x=w86, y=0) -> (max(x,y)=w83:dbl)  [unwired: 1 out]
        n86 = local read "DESD2 SOC"() -> (w106:dbl)
        n87 = Boolean Array To Number(Boolean array=w129) -> (number=w79:u32)
        n88 = local read "DESD1 SOC"() -> (w117:dbl)
        n89 = Max & Min(x=w102, y=255) -> (min(x,y)=w93:dbl)  [unwired: 1 out]
        n90 = Max & Min(x=w97, y=0) -> (max(x,y)=w94:dbl)  [unwired: 1 out]
        n91 = Max & Min(x=w113, y=255) -> (min(x,y)=w104:dbl)  [unwired: 1 out]
        n92 = Max & Min(x=w124, y=255) -> (min(x,y)=w115:dbl)  [unwired: 1 out]
        n93 = Max & Min(x=w108, y=0) -> (max(x,y)=w105:dbl)  [unwired: 1 out]
        n94 = Max & Min(x=w119, y=0) -> (max(x,y)=w116:dbl)  [unwired: 1 out]
        n95 = Bundle "WT Command Cluster"("192.168.10.81", "wind speed"=w125, w126, w126, w126, w126) -> (w76:T3)  [unwired: 1 in]
        n96 = Build Array("IO 9", "IO 10", "IO 11", "IO 12", "IO 13", "IO 14", "IO 15", "IO 16") -> (w130:bool[])
        n97 = Bundle "DESD4 Command Cluster"("192.168.10.54", "DESD4 SOC"=w84, w83, w82, w81, w81) -> (w72:T4)  [unwired: 1 in]
        n98 = Boolean Array To Number(Boolean array=w130) -> (number=w78:u32)
        n99 = Bundle "IO Command Cluster"("192.168.10.91", w79, w78, w77, w77, w77) -> (w71:cluster{string, u32, u32, i32, i32, i32})  [unwired: 1 in]
        n100 = Bundle "DESD3 Command Cluster"("192.168.10.53", "DESD3 SOC"=w95, w94, w93, w92, w92) -> (w73:T5)  [unwired: 1 in]
        n101 = Bundle "DESD2 Command Cluster"("192.168.10.52", "DESD2 SOC"=w106, w105, w104, w103, w103) -> (w74:T6)  [unwired: 1 in]
        n102 = Bundle "DESD1 Command Cluster"("192.168.10.51", "DESD1 SOC"=w117, w116, w115, w114, w114) -> (w75:T7)  [unwired: 1 in]
        n103 = Build Array(w76, w75, w74, w73, w72, w71) -> (w70:T8)
        n104 = for {
          tunnel: w70 -> [w153] mode=indexing
          n105 = Unbundle(w153) -> (w152:string, "DESD4 SOC"=w151:dbl, w150:dbl, w149:dbl, w148:i32, w147:i32)
          n106 = call "SendUDP.vi"("Arg3"=w151, "IP"=w152, "Port"=8008, "Arg4"=w150, "Arg5"=w149, "Arg6"=w148, "Arg7"=w147) -> ()  [unwired: 9 in]
        }
      }
      event "BTN_Wind_Turbine": Value Change {
        n107 = event-data() -> ()  [unwired: 1 in, 6 out]
        n108 = local write "Device Name"("WT 1 — Wind Turbine") -> ()
        n109 = local write "Device Badge"("weather input") -> ()
        n110 = local write "Selected Summary"("Selected: WT 1") -> ()
        n111 = local write "Device Description"("P_min = 0 MW, P_max = 1.05 MW") -> ()
      }
      event "5-Day Rainstorm-to-Flood": Value Change {
        n112 = event-data() -> ()  [unwired: 1 in, 6 out]
        n113 = Read from Text File(file (use dialog)=path "D:/learn/led_test.txt") -> (text=w159:string)  [unwired: 3 in, 3 out]
        n114 = while {
          shift-right: [w164] -> _
          shift-left: w159 -> [w165]
          stop <- w163 stop-if-true
          n115 = Match Pattern(string=w165, regular expression="\\n") -> (before substring=w162:string, after substring=w164:string)  [unwired: 1 in, 2 out]
          n116 = call <vilib>:"Trim Whitespace.vi"("string"=w162) -> ("trimmed string"=w170:string)  [unwired: 1 in]
          n117 = Match Pattern(string=w162, regular expression="#") -> (before substring=w172:string)  [unwired: 1 in, 3 out]
          n118 = String Length(string=w170) -> (length=w169:i32)
          n119 = Equal To 0?(x=w169) -> (x = 0?=w167:bool)
          n120 = Equal?(x=w172, y="" ("regular expression")) -> (x = y?=w168:bool)
          n121 = Or(x=w168, y=w167) -> (x .or. y?=w166:bool)
          n122 = case shown="False" w166 {
            tunnel: w162 -> [w189 _]
            frame False {
              n123 = Scan From String(format string="%d %d %d %d %d %d | %d" ("regular expression"), input string=w189) -> (output 1=w187:i32, output 2=w181:u8, output 3=w180:u8, output 4=w179:u8, output 5=w178:u8, output 6=w177:u8, output 7=w176:i32)  [unwired: 9 in, 3 out]
              n124 = Wait (ms)(milliseconds to wait=w176) -> ()  [unwired: 1 out]
              n125 = Add(x=w187, y=0) -> (x+y=w186:i32)
              n126 = Format Into String(format string="192.168.10.%d", w186) -> (resulting string=w184:string)  [unwired: 2 in, 1 out]
              n127 = call "SendUDP.vi"("Arg3"=w181, "IP"=w184, "Port"=8008, "Arg4"=w180, "Arg5"=w179, "Arg6"=w178, "Arg7"=w177) -> ()  [unwired: 9 in]
            }
            frame True {
            }
          }
          n128 = String Length(string=w164) -> (length=w174:i32)
          n129 = Equal To 0?(x=w174) -> (x = 0?=w163:bool)
          n130 = local write "5-Day Rainstorm-to-Flood"(FALSE) -> ()
          n131 = local write "script Status"(w162) -> ()
        }
      }
      event "stop": Value Change {
        n132 = event-data() -> ()  [unwired: 1 in, 6 out]
      }
    }
  }
